vi "INL_Measurement_Spec.vi"(0 "Start Value":dbl, 1 "Resolution":u16, 5 "Stop Value":dbl, 7 "Step Size":dbl, 9 "Settling Time":u32, 11 "Error In":errorcluster, 12 "Reference Voltage":dbl format="%.2p") -> (15 "Error Out":errorcluster)   [LabVIEW 2026, in "Core.lvlib"]
doc: "This VI allows the user to configure the specifications required for the given test [INL]"
uses:
  Core.lvlib
  TypeDefs/Enum_Events.ctl
  TypeDefs/Enum_Notifier_Name.ctl
  TypeDefs/Enum_Notifier_Options.ctl
  TypeDefs/Notification_Clusters/Cluster_INL_Measurement_Specs.ctl
  TypeDefs/Enum_Event_Options.ctl
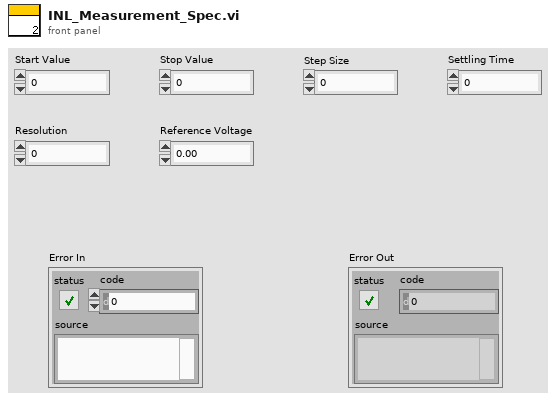
[diagram p1: front panel]
types:
  T1 = typedef "Core.lvlib/Enum_Events.ctl" = enum16{"Stop All", "Stop Subpanel", "Stop Test Spec", "Stop Result"}
  T2 = typedef "Core.lvlib/Enum_Event_Options.ctl" = enum16{"Create", "Generate", "Event Ref", "Destroy"}
  T3 = typedef "Core.lvlib/Cluster_INL_Measurement_Specs.ctl" = cluster{" Resolution":u16, "Reference Voltage":dbl, "Settling Time":u32, "Start":dbl, "Step Size":dbl, "Stop":dbl}
  T4 = typedef "Core.lvlib/Enum_Notifier_Options.ctl" = enum16{"Create", "Send", "Status", "Release"}
  T5 = typedef "Core.lvlib/Enum_Notifier_Name.ctl" = enum16{"Device Type", "Test", "Instrument Spec", "Measurement Spec"}
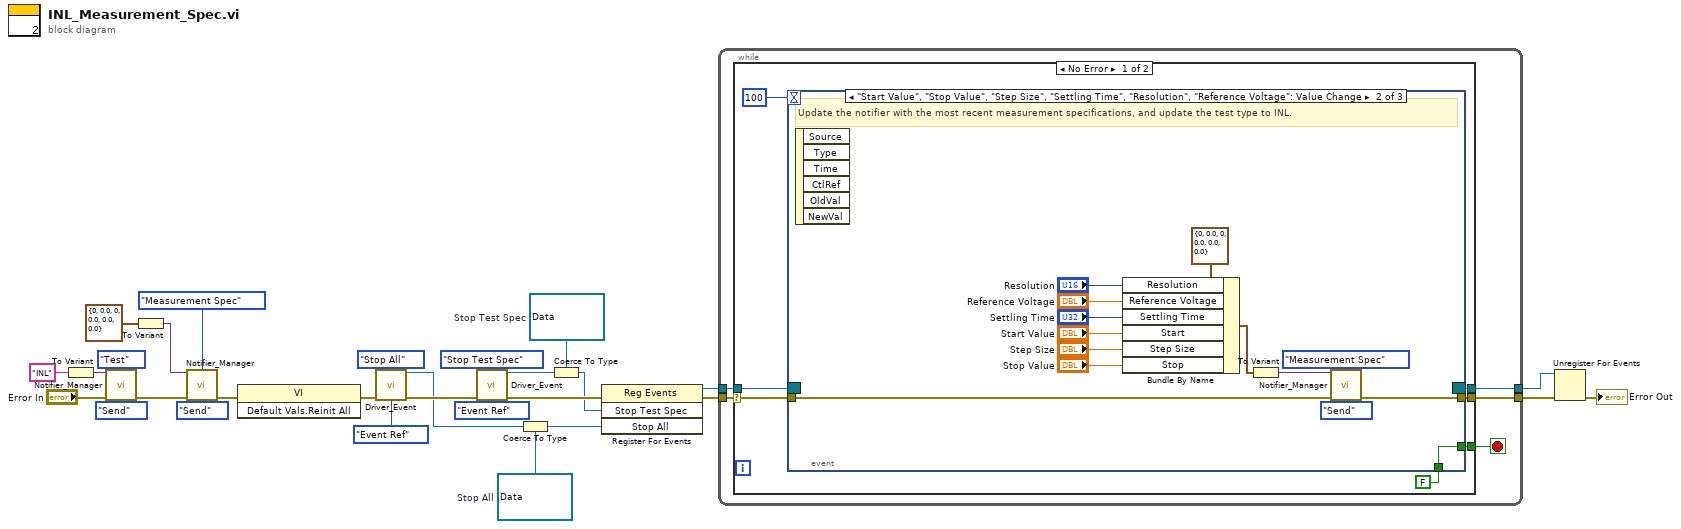
[diagram p0: block diagram]
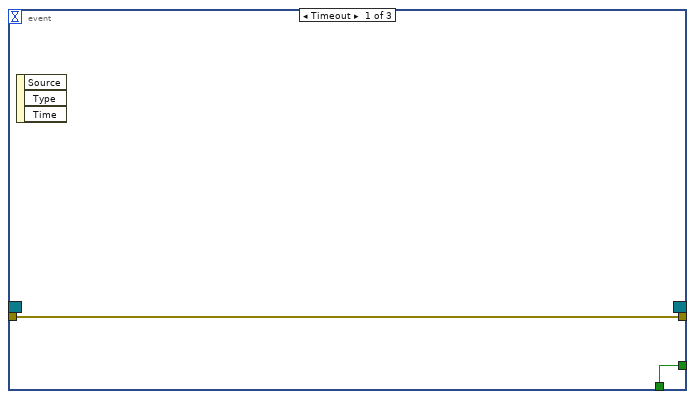
[diagram p2: hidden frame]
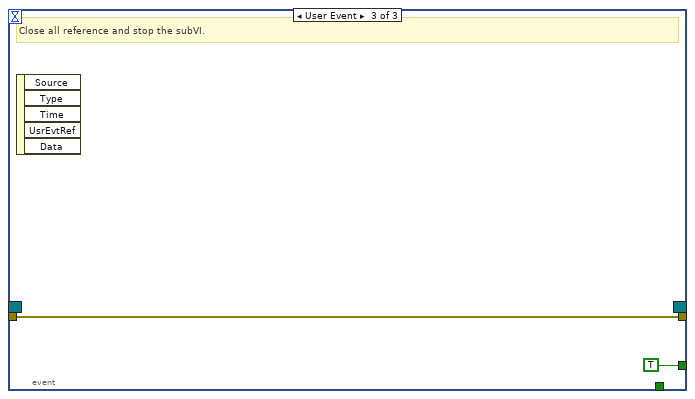
[diagram p3: hidden frame]
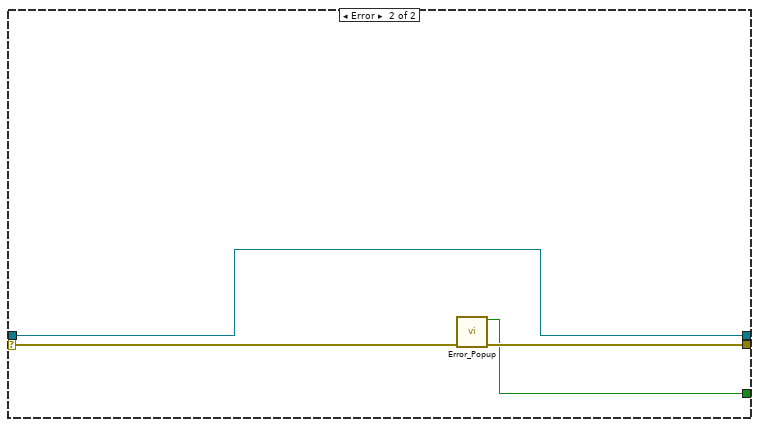
[diagram p4: hidden frame]
diagram:
  w1 = refnum<user-event> refnum  # Stop All
  w21 = refnum<user-event> refnum  # Stop Test Spec
  n1 = To Variant(anything="INL") -> (Variant=w18:variant)
  n2 = call "Notifier_Manager.vi"("Notifier Data"=w18, "Notifier Name"=Enum_Notifier_Name."Test", "Error In"="Error In", "Notifier Options"=Enum_Notifier_Options."Send") -> ("Error Out"=w12:errorcluster)  [unwired: 10 in, 1 out]
  n3 = To Variant(anything=T3 {" Resolution"=0, "Reference Voltage"=0.0, "Settling Time"=0, "Start"=0.0, "Step Size"=0.0, "Stop"=0.0} ("Measurement Specs")) -> (Variant=w8:variant)
  n4 = call "Notifier_Manager.vi"("Notifier Data"=w8, "Notifier Name"=Enum_Notifier_Name."Measurement Spec", "Error In"=w12, "Notifier Options"=Enum_Notifier_Options."Send") -> ("Error Out"=w13:errorcluster)  [unwired: 10 in, 1 out]
  n5 = invoke class="VI" method="Default Vals.Reinit All"(error in=w13) -> (error out=w7:errorcluster)  [unwired: 2 in, 2 out]
  n6 = call "Driver_Event.vi"("Event"=Enum_Events."Stop All", "Error In"=w7, "Event Operation"=Enum_Event_Options."Event Ref") -> ("Event Ref"=w3:refnum<user-event>, "Error Out"=w6:errorcluster)  [unwired: 11 in]
  n7 = call "Driver_Event.vi"("Event"=Enum_Events."Stop Test Spec", "Error In"=w6, "Event Operation"=Enum_Event_Options."Event Ref") -> ("Event Ref"=w28:refnum<user-event>, "Error Out"=w27:errorcluster)  [unwired: 11 in]
  n8 = Coerce To Type(0:w3, 1:w1) -> (2:w2:refnum<user-event>)
  n9 = Coerce To Type(0:w28, 1:w21) -> (2:w22:refnum<user-event>)
  n10 = register-events(error in=w27, w22, w2) -> (reference out=w25:refnum<event-registration>, error out=w26:errorcluster)  [unwired: 1 in]
  n11 = while {
    tunnel: w26 -> [w33]
    tunnel: [w34] -> w29
    tunnel: w25 -> [w32]
    tunnel: [w31] -> w23
    stop <- w30 stop-if-true
    n12 = case shown="No Error" w33 {
      selector: w33 -> [w40 w63]
      tunnel: [w41 w62] -> w34
      tunnel: w32 -> [w38 w61]
      tunnel: [w37 w61] -> w31
      tunnel: [w36 w60] -> w30
      frame No Error {
        n13 = event shown="[1] \"Start Value\", \"Stop Value\", \"Step Size\", \"Settling Time\", \"Resolution\", \"Reference Voltage\": Value Change" {
          selector: w38 -> [_ _ _]
          dyn-events: [_ _ _] -> w37
          timeout: 100 -> [_ _ _]
          tunnel: [w43 w44 w58] -> w41
          tunnel: w40 -> [w43 w56 w58]
          tunnel: [w42 w57 TRUE] -> w36
          tunnel: FALSE -> [w42 w57 _]
          event Timeout {
            n14 = event-data() -> ()  [unwired: 1 in, 3 out]
          }
          event "Start Value", "Stop Value", "Step Size", "Settling Time", "Resolution", "Reference Voltage": Value Change {
            # "Update the notifier with the most recent measurement specifications, and update the test type to INL."
            n15 = event-data() -> ()  [unwired: 1 in, 6 out]
            n16 = Bundle By Name(cluster=T3 {" Resolution"=0, "Reference Voltage"=0.0, "Settling Time"=0, "Start"=0.0, "Step Size"=0.0, "Stop"=0.0} ("Measurement Specs"), "Resolution"="Resolution", "Reference Voltage"="Reference Voltage", "Settling Time"="Settling Time", "Start"="Start Value", "Step Size"="Step Size", "Stop"="Stop Value") -> (w46:T3)
            n17 = To Variant(anything=w46) -> (Variant=w45:variant)
            n18 = call "Notifier_Manager.vi"("Notifier Data"=w45, "Notifier Name"=Enum_Notifier_Name."Measurement Spec", "Error In"=w56, "Notifier Options"=Enum_Notifier_Options."Send") -> ("Error Out"=w44:errorcluster)  [unwired: 10 in, 1 out]
          }
          event User Event {
            # "Close all reference and stop the subVI."
            n19 = event-data() -> ()  [unwired: 1 in, 5 out]
          }
        }
      }
      frame Error {
        n20 = call "Error_Popup.vi"("Error In"=w63) -> ("Stop?"=w60:bool, "Error Out"=w62:errorcluster)  [unwired: 13 in]
      }
    }
  }
  n21 = Unregister For Events(event registration refnum=w23, error in=w29) -> (error out=→"Error Out":errorcluster)
